vi "Func - LV runtime error handler (Error Cluster).vi"(5 "InstanceRef":T1, 6 "error in":bool, 7 "Gen CE error?":bool, 9 "LabVIEW error":errorcluster) -> (0 "error out":bool, 2 "LV error code":i32, 3 "dup LabVIEW error":errorcluster, 4 "LV error status":bool)   [LabVIEW 2021]
doc: "This VI handles errors returned by LabVIEW VIs and functions. Refer to the VI help for more details.\n\n::: CalcExpress Toolkit :::\nCopyright (c) 2000-2026 Konstantin Shifershteyn. All rights reserved."
uses:
  cetypes.llb/CalcExpress Instance RefNum.ctl
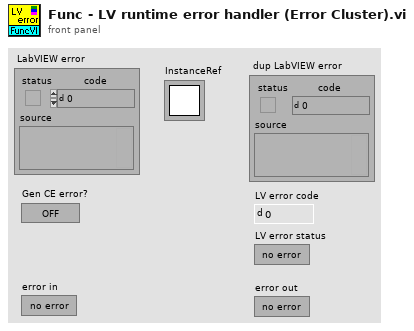
[diagram p1: front panel]
types:
  T1 = typedef "CalcExpress Instance RefNum.ctl" = refnum<k1>
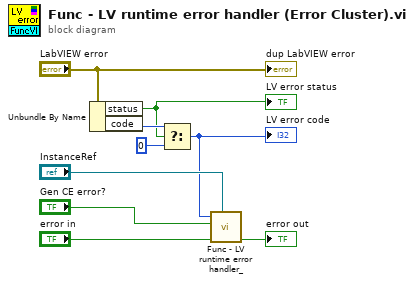
[diagram p0: block diagram]
diagram:
  n1 = Unbundle By Name("LabVIEW error") -> ("status"=w1:bool, "code"=w4:i32)
  "LV error status" <- w1
  n2 = Select(t=w4, s=w1, f=0) -> (s? t:f=w2:i32)
  "LV error code" <- w2
  n3 = call "Func - LV runtime error handler_.vi"("InstanceRef"="InstanceRef", "error in"="error in", "Gen CE error?"="Gen CE error?", "LabVIEW error code"=w2) -> ("error out"=→"error out":bool)  [unwired: 7 in]
  "dup LabVIEW error" <- "LabVIEW error"
